vi "VIH ProjFile - Item Rule Array - Read.vi"(7 "Project Folder":path, 8 "error in":errorcluster, 11 "XML Parent Item":refnum<k20>) -> (0 "error out":errorcluster, 1 "Item Rules":T1[](array[typedef]), 2 "Item Paths":path[](array[path]), 3 "dup XML Parent Item":refnum<k20>)   [LabVIEW 2014]
doc: "::: VI Helpeks :::\nCopyright (c) 2000-2026 Konstantin Shifershteyn. All rights reserved."
uses:
  _VIH HelpGen.llb/VIH HelpGen Typedef - Cluster - File Rule.ctl
  _VIH HelpGen.llb/VIH HelpGen Typedef - Enum - Default,Enable,Disable.ctl
  _VIH HelpGen.llb/VIH HelpGen Typedef - Cluster - File Rule - Source Paths.ctl
  _VIH HelpGen.llb/VIH HelpGen Typedef - Cluster - File Rule - Target Paths.ctl
  _VIH HelpGen.llb/VIH HelpGen Typedef - Enum - Description Mode.ctl
  _VIH HelpGen.llb/VIH HelpGen Typedef - Cluster - Control Rule.ctl
  _VIH HelpGen.llb/VIH HelpGen Typedef - Cluster - Enum Value Info.ctl
  _VIH HelpGen.llb/VIH HelpGen Typedef - Cluster - Group Rule - Flags.ctl
  <vilib>/xml/Close Reference(Node).vi
  <vilib>/xml/NI_XML.lvlib
panel:
  # "VI Helpeks\nCopyright (c) 2012-2026 Konstantin Shifershteyn"
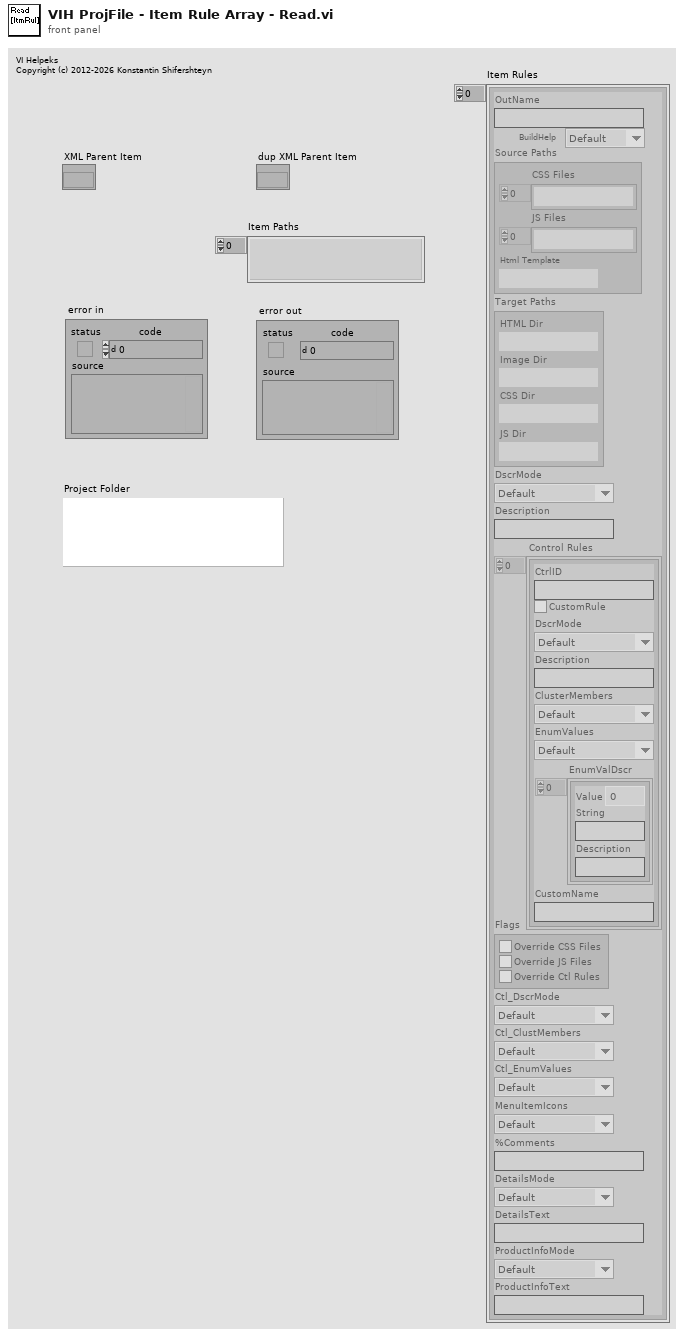
[diagram p1: front panel]
types:
  T1 = typedef "VIH HelpGen Typedef - Cluster - File Rule.ctl" = cluster{"OutName":string, "BuildHelp":T2, "Source Paths":T3, "Target Paths":T4, "DscrMode":T5, "Description":string, "Control Rules":T6[], "Flags":T8, "Ctl_DscrMode":T5, "Ctl_ClustMembers":T2, "Ctl_EnumValues":T2, "MenuItemIcons":T2, "%Comments":string, "DetailsMode":T5, "DetailsText":string, "ProductInfoMode":T2, "ProductInfoText":string}
  T2 = typedef "VIH HelpGen Typedef - Enum - Default,Enable,Disable.ctl" = enum16{"Default", "Enable", "Disable"}
  T3 = typedef "VIH HelpGen Typedef - Cluster - File Rule - Source Paths.ctl" = cluster{"CSS Files":path[], "JS Files":path[], "Html Template":path}
  T4 = typedef "VIH HelpGen Typedef - Cluster - File Rule - Target Paths.ctl" = cluster{"HTML Dir":path, "Image Dir":path, "CSS Dir":path, "JS Dir":path}
  T5 = typedef "VIH HelpGen Typedef - Enum - Description Mode.ctl" = enum16{"Default", "Description", "Description1", "Description2", "Custom", "None"}
  T6 = typedef "VIH HelpGen Typedef - Cluster - Control Rule.ctl" = cluster{"CtrlID":string, "CustomRule":bool, "DscrMode":T5, "Description":string, "ClusterMembers":T2, "EnumValues":T2, "EnumValDscr":T7[], "CustomName":string}
  T7 = typedef "VIH HelpGen Typedef - Cluster - Enum Value Info.ctl" = cluster{"Value":ext, "String":string, "Description":string}
  T8 = typedef "VIH HelpGen Typedef - Cluster - Group Rule - Flags.ctl" = cluster{"Override CSS Files":bool, "Override JS Files":bool, "Override Ctl Rules":bool}
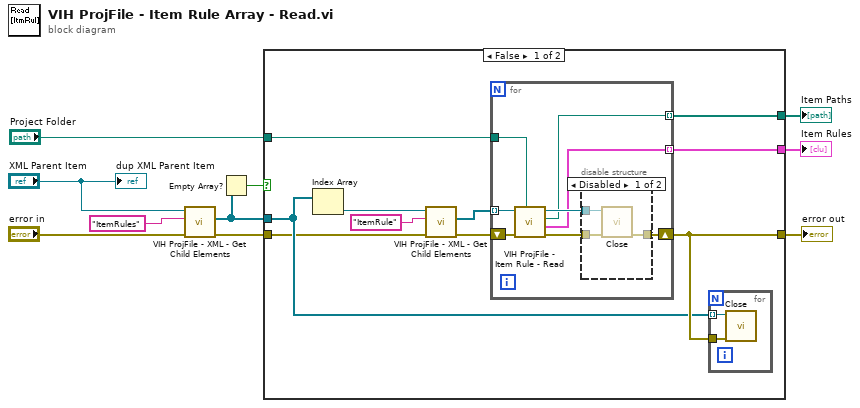
[diagram p0: block diagram]
diagram:
  n1 = call "VIH ProjFile - XML - Get Child Elements.vi"("error in"="error in", "Tag Name"="ItemRules", "XML Parent Item"="XML Parent Item") -> ("error out"=w5:errorcluster, "Array of Elements"=w4:refnum<k20>[])  [unwired: 6 in, 1 out]
  n2 = Empty Array?(array=w4) -> (empty?=w7:bool)
  n3 = case shown="False" w7 {
    tunnel: [w20 _] -> w10
    tunnel: [w19 _] -> w9
    tunnel: w5 -> [w15 w35]
    tunnel: [w18 w35] -> w8
    tunnel: w4 -> [w17 _]
    tunnel: "Project Folder" -> [w16 _]
    frame False {
      n4 = Index Array(array=w17) -> (element=w14:refnum<k20>)  [unwired: 1 in]
      n5 = call "VIH ProjFile - XML - Get Child Elements.vi"("error in"=w15, "Tag Name"="ItemRule", "XML Parent Item"=w14) -> ("error out"=w12:errorcluster, "Array of Elements"=w11:refnum<k20>[])  [unwired: 6 in, 1 out]
      n6 = for {
        shift-right: [w26] -> w18
        shift-left: w12 -> [w30]
        tunnel: w11 -> [w29] mode=indexing
        tunnel: [w25] -> w20 mode=indexing
        tunnel: [w24] -> w19 mode=indexing
        tunnel: w16 -> [w23]
        n7 = call "VIH ProjFile - Item Rule - Read.vi"("Project Folder"=w23, "error in"=w30, "XML Item"=w29) -> ("error out"=w28:errorcluster, "Item Rule out"=w24:T1, "Item Path"=w25:path, "dup XML Item"=w27:refnum<k20>)  [unwired: 5 in]
        n8 = disable-structure shown="Disabled" {
          disable-tunnel: w28 -> [w33 w34]
          disable-tunnel: w27 -> [w32 _]
          disable-tunnel: [w31 w34] -> w26
          frame Disabled {
            n9 = call-poly <vilib>:"Close.vi"("error in (no error)"=w33, "node"=w32) -> ("error out"=w31:errorcluster)  [unwired: 7 in]
          }
          frame Enabled {
          }
        }
      }
      n10 = for {
        tunnel: w17 -> [w22] mode=indexing
        tunnel: w18 -> [w21]
        n11 = call-poly <vilib>:"Close.vi"("error in (no error)"=w21, "node"=w22) -> ()  [unwired: 7 in, 1 out]
      }
    }
    frame True {
    }
  }
  "error out" <- w8
  "Item Paths" <- w10
  "Item Rules" <- w9
  "dup XML Parent Item" <- "XML Parent Item"
